vi "ApplyPropertyTemplateToMethod.vi"(0 "ClassWriterNative in":refnum<class "ClassWriterNative.lvclass">, 1 "VIRef":refnum<vi>, 2 "ClassRef":refnum<vi>, 3 "PropertyName":string, 4 "MethodTemplateName":string, 5 "error in (no error)":errorcluster) -> (14 "ClassWriterNative out":refnum<class "ClassWriterNative.lvclass">, 19 "error out":errorcluster)   [LabVIEW 2020, in "ClassWriterNative.lvclass"]
uses:
  ClassWriterNative.lvclass
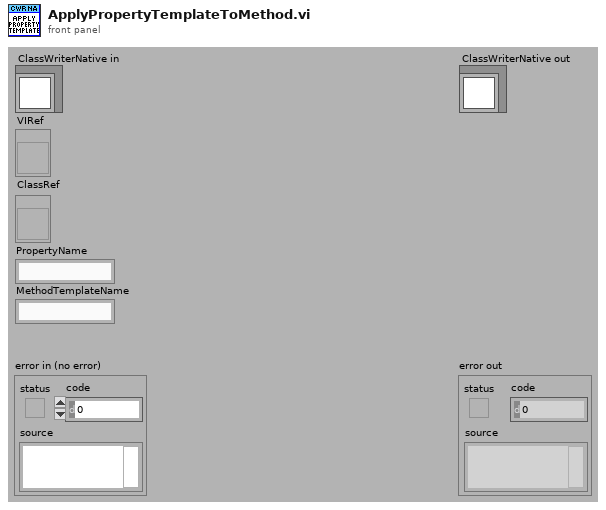
[diagram p1: front panel]
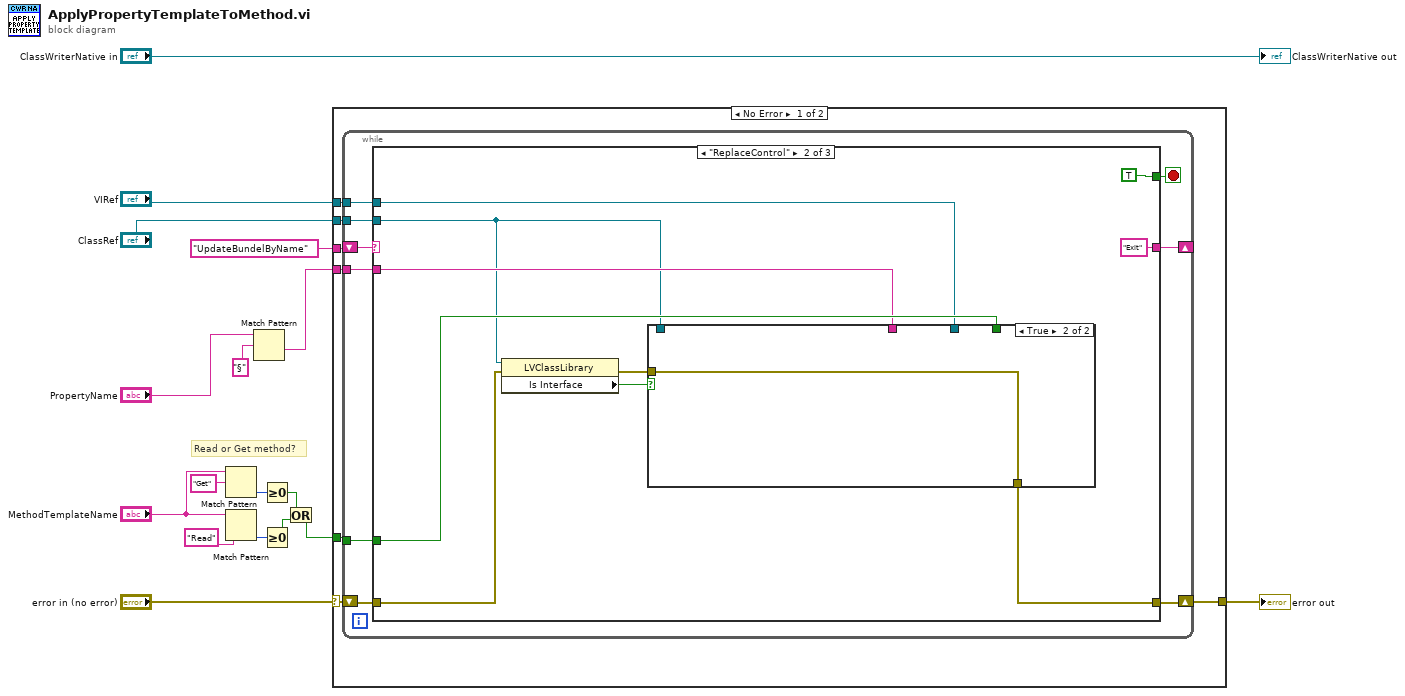
[diagram p0: block diagram]
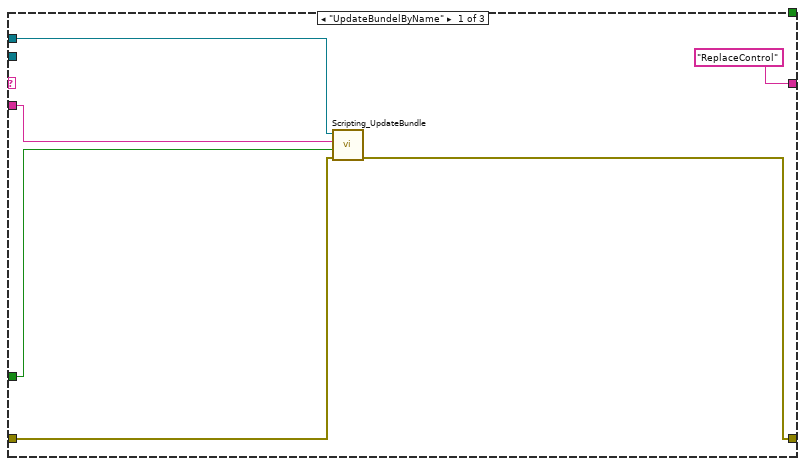
[diagram p2: hidden frame]
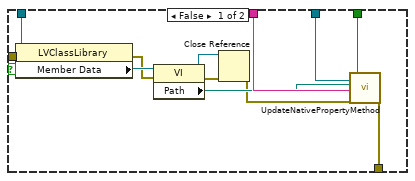
[diagram p3: hidden frame]
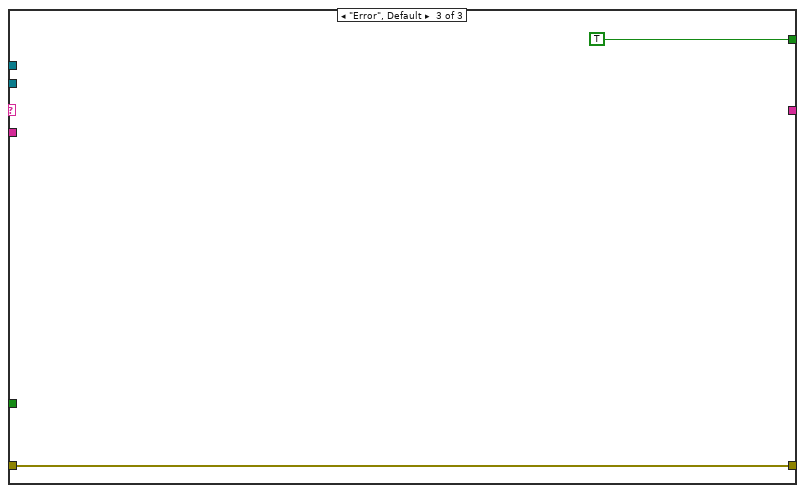
[diagram p4: hidden frame]
diagram:
  # "Read or Get method?"
  n1 = Match Pattern(string="MethodTemplateName", regular expression="Get") -> (offset past match=w5:i32)  [unwired: 1 in, 3 out]
  n2 = Match Pattern(string="MethodTemplateName", regular expression="Read") -> (offset past match=w16:i32)  [unwired: 1 in, 3 out]
  n3 = Match Pattern(string="PropertyName", regular expression="§" ("search string")) -> (after substring=w8:string)  [unwired: 1 in, 3 out]
  n4 = Greater Or Equal To 0?(x=w5) -> (x >= 0?=w3:bool)
  n5 = Greater Or Equal To 0?(x=w16) -> (x >= 0?=w4:bool)
  n6 = Or(x=w3, y=w4) -> (x .or. y?=w2:bool)
  n7 = case shown="No Error" "error in (no error)" {
    selector: "error in (no error)" -> [w18 w65]
    tunnel: "UpdateBundelByName" -> [w24 _]
    tunnel: "VIRef" -> [w23 _]
    tunnel: "ClassRef" -> [w22 _]
    tunnel: w2 -> [w21 _]
    tunnel: w8 -> [w20 _]
    tunnel: [w19 w65] -> w13
    frame No Error {
      n8 = while {
        tunnel: w23 -> [w33]
        tunnel: w20 -> [w32]
        shift-right: [w30] -> w19
        shift-left: w18 -> [w31]
        shift-right: [w28] -> _
        shift-left: w24 -> [w29]
        tunnel: w22 -> [w26]
        tunnel: w21 -> [w25]
        stop <- w27 stop-if-true
        n9 = case shown="\"ReplaceControl\"" w29 {
          tunnel: w33 -> [w35 w45 _]
          tunnel: w32 -> [w37 w44 _]
          tunnel: w31 -> [w36 w42 w63]
          tunnel: [w39 w47 w63] -> w30
          tunnel: ["ReplaceControl" "Exit" _] -> w28
          tunnel: [_ TRUE TRUE] -> w27
          tunnel: w26 -> [_ w43 _]
          tunnel: w25 -> [w34 w46 _]
          frame "UpdateBundelByName" {
            n10 = call "Scripting_UpdateBundle.vi"("error in (no error)"=w36, "Boolean"=w34, "PropertyName"=w37, "VI in"=w35) -> ("error out"=w39:errorcluster)  [unwired: 7 in]
          }
          frame "ReplaceControl" {
            n11 = property class="LVClassLibrary"(reference=w43, error in=w42) -> (error out=w41:errorcluster, "Is Interface"=w40:bool)  [unwired: 1 out]
            n12 = case shown="True" w40 {
              tunnel: [w61 w62] -> w47
              tunnel: w46 -> [w60 _]
              tunnel: w45 -> [w59 _]
              tunnel: w44 -> [w58 _]
              tunnel: w43 -> [w51 _]
              tunnel: w41 -> [w50 w62]
              frame False {
                n13 = property class="LVClassLibrary"(reference=w51, error in=w50) -> (error out=w56:errorcluster, "Member Data"=w57:refnum<vi>)  [unwired: 1 out]
                n14 = property class="VI"(reference=w57, error in=w56) -> (reference out=w54:refnum<vi>, error out=w55:errorcluster, "Path"=w53:path)
                n15 = Close Reference(reference=w54, error in (no error)=w55) -> (error out=w52:errorcluster)
                n16 = call "UpdateNativePropertyMethod.vi"("VI"=w59, "TypeDefControl"=w53, "Property"=w58, "error IO"=w52, "GetMethod"=w60) -> ("error out"=w61:errorcluster)  [unwired: 14 in]
              }
              frame True {
              }
            }
          }
          frame "Error", Default {
          }
        }
      }
    }
    frame Error {
    }
  }
  "error out" <- w13
  "ClassWriterNative out" <- "ClassWriterNative in"
